vi "Sync To Server.vi"(8 "error in (no error)":errorcluster, 9 "Station":string="LTS-01", 10 "Connection String":string="Provider=MSOLEDBSQL;Data Source=.\\SQLEXPRESS;Initial Catalog=LTS;Integrated Security=SSPI;TrustServerCertificate=Yes;", 11 "DB Path":path) -> (0 "error out":errorcluster, 3 "Runs Synced":i32)   [LabVIEW 2026]
uses:
  <vilib>/drjdpowell/SQLite Library/SQL Connection/Open (path).vi
  <vilib>/drjdpowell/SQLite Library/SQL Connection/Open (string).vi
  <vilib>/AdvancedString/Path To Command Line String.vi
  <vilib>/drjdpowell/SQLite Library/SQL Connection/Execute SQL.vi
  <vilib>/addons/database/Connection.llb/DB Tools Open Connec (String).vi
  <vilib>/addons/database/Command.llb/Cmd Set Parameter Value (C).vi
  <vilib>/addons/database/Command.llb/Cmd Execute.vi
  <vilib>/addons/database/Recordset.llb/Rec Fetch Recordset Data (CR).vi
  <vilib>/addons/database/Recordset.llb/Rec Destroy - Command.vi
  <vilib>/drjdpowell/SQLite Library/SQL Connection/Execute SQL (No results).vi
  <vilib>/addons/database/Command.llb/Cmd Delete.vi
  <vilib>/drjdpowell/SQLite Library/SQL Connection/Connection.lvclass
  <vilib>/drjdpowell/SQLite Library/SQLite.lvlib
  <vilib>/addons/database/NI_Database_API.lvlib
panel:
  out "Result Set":string[][](table) caption="Result Set (from first statement with results)"
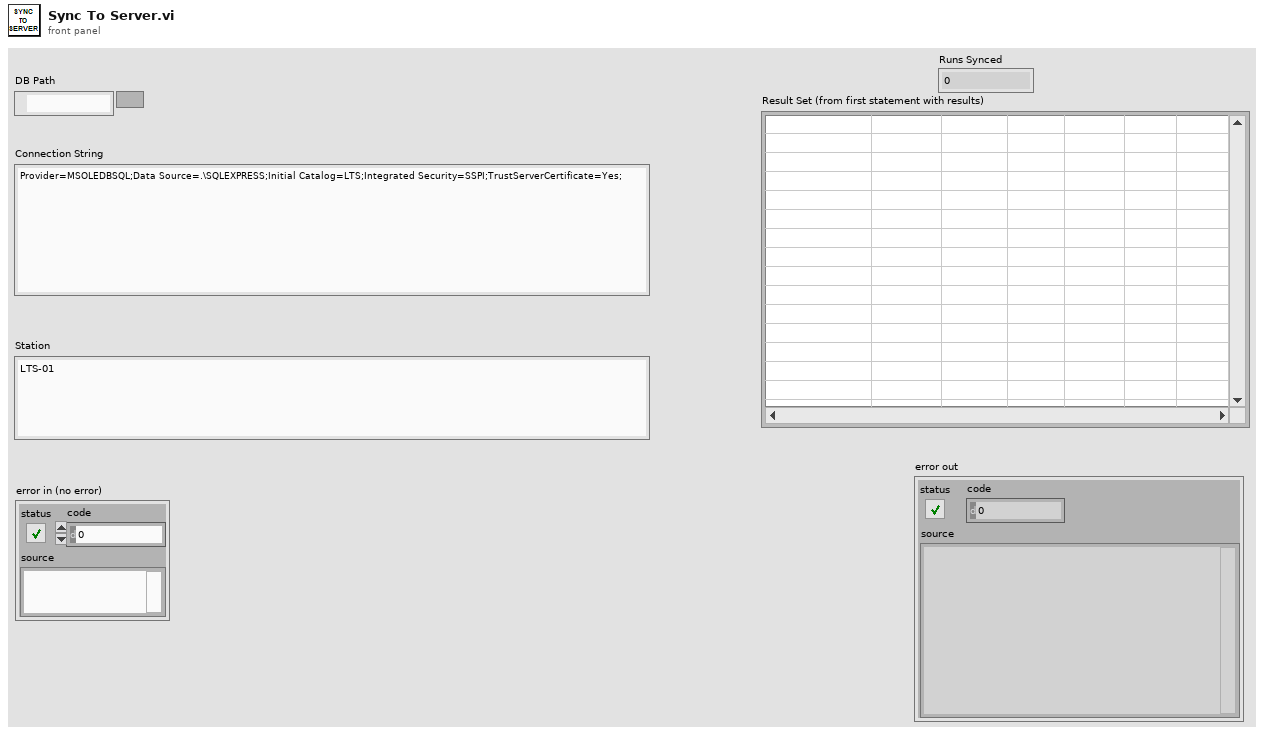
[diagram p1: front panel]
types:
  T1 = typedef "NI_Database_API.lvlib/Conn ObjectReference.ctl" = refnum<k1>
  T2 = typedef "NI_Database_API.lvlib/Cmd ObjectReference.ctl" = refnum<k1>
  T3 = typedef "NI_Database_API.lvlib/Cmd-Rec Object Reference.ctl" = refnum<k1>
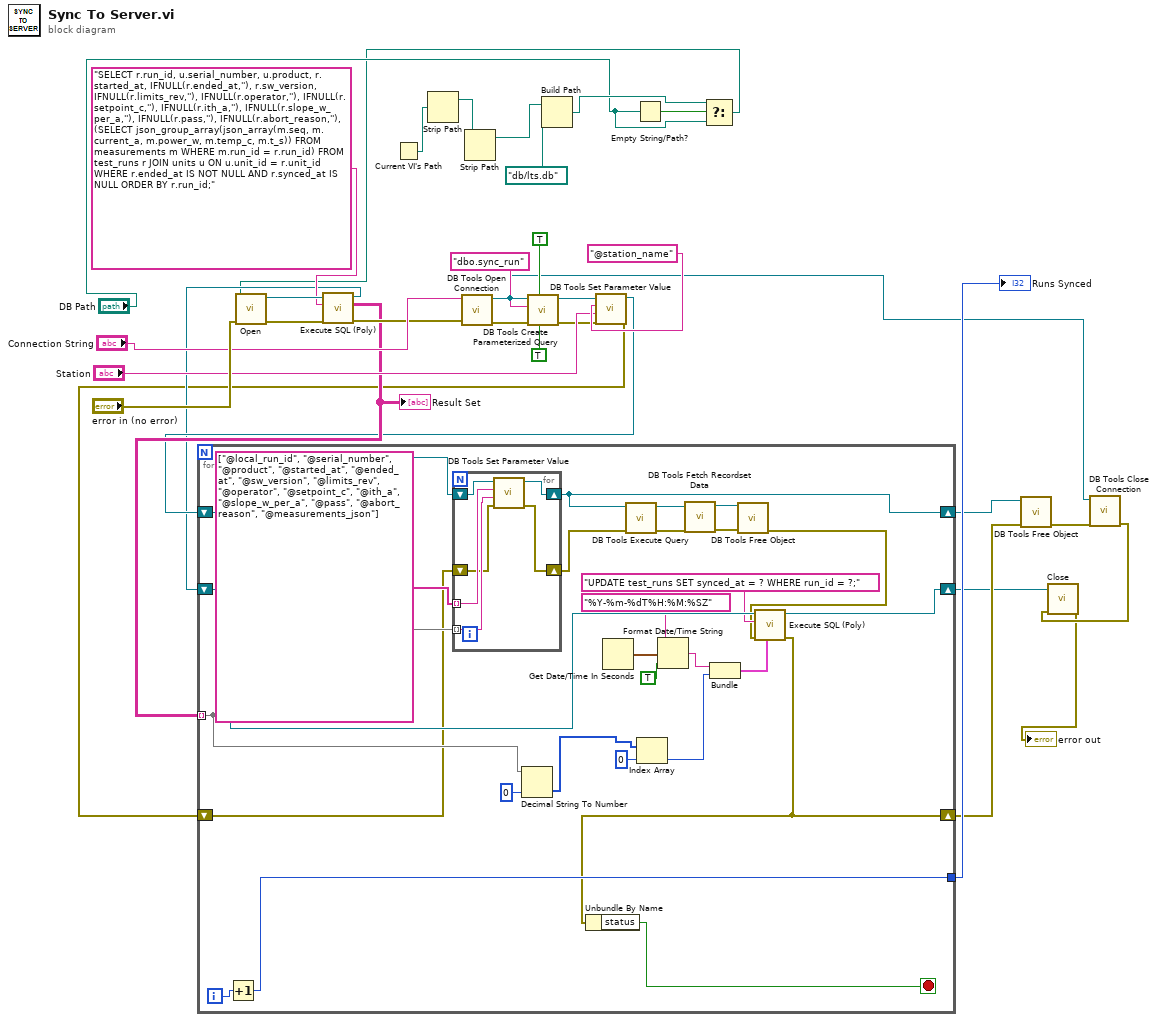
[diagram p0: block diagram]
diagram:
  n1 = Current VI's Path() -> (path=w8:path)
  n2 = Strip Path(path=w8) -> (stripped path=w7:path)  [unwired: 1 out]
  n3 = Strip Path(path=w7) -> (stripped path=w6:path)  [unwired: 1 out]
  n4 = Build Path(base path=w6, name or relative path=path "db/lts.db") -> (appended path=w3:path)
  n5 = Empty String/Path?(string/path="DB Path") -> (empty?=w4:bool)
  n6 = Select(t=w3, s=w4, f="DB Path") -> (s? t:f=w1:path)
  n7 = call-poly <vilib>:"Open.vi"("error in (no error)"="error in (no error)", "db file"=w1) -> ("error out"=w24:errorcluster, "SQLite Connection"=w33:refnum<class "Connection.lvclass">)  [unwired: 8 in]
  n8 = call-poly <vilib>:"Execute SQL (Poly).vi"("error in (no error)"=w24, "SQL"="SELECT r.run_id, u.serial_number, u.product, r.started_at, IFNULL(r.ended_at,''), r.sw_version, IFNULL(r.limits_rev,''), IFNULL(r.operator,''), IFNULL(r.setpoint_c,''), IFNULL(r.ith_a,''), IFNULL(r.slope_w_per_a,''), IFNULL(r.pass,''), IFNULL(r.abort_reason,''), (SELECT json_group_array(json_array(m.seq, m.current_a, m.power_w, m.temp_c, m.t_s)) FROM measurements m WHERE m.run_id = r.run_id) FROM test_runs r JOIN units u ON u.unit_id = r.unit_id WHERE r.ended_at IS NOT NULL AND r.synced_at IS NULL ORDER BY r.run_id;", "SQLite Connection in"=w33) -> ("error out"=w23:errorcluster, "Result Set"=w20:string[][], "SQLite Connection"=w18:refnum<class "Connection.lvclass">)  [unwired: 5 in, 1 out]
  "Result Set" <- w20
  n9 = call-poly <vilib>:"DB Tools Open Connection.vi"("error in (no error)"=w23, "connection information"="Connection String") -> ("error out"=w22:errorcluster, "connection reference"=w13:T1)  [unwired: 6 in]
  n10 = call <vilib>:"DB Tools Create Parameterized Query.vi"("stored procedure? (F)"=TRUE, "auto-detect parameters? (F)"=TRUE, "error in (no error)"=w22, "SQL query"="dbo.sync_run", "connection reference"=w13) -> ("error out"=w21:errorcluster, "command reference"=w27:T2)  [unwired: 2 in, 1 out]
  n11 = call-poly <vilib>:"DB Tools Set Parameter Value.vi"("error in (no error)"=w21, "value"="Station", "parameter index"="@station_name", "command reference"=w27) -> ("error out"=w17:errorcluster, "command reference out"=w19:T2)  [unwired: 4 in]
  n12 = for {
    tunnel: w20 -> [w39] mode=indexing
    shift-right: [w58] -> w9
    shift-left: w19 -> [w60]
    shift-right: [w40] -> w12
    shift-left: w18 -> [w53]
    shift-right: [w35] -> w15
    shift-left: w17 -> [w36]
    tunnel: [w41] -> w16
    i -> [w42]
    stop <- w59 stop-if-true
    n13 = Increment(x=w42) -> (x+1=w41:i32)
    n14 = for {
      tunnel: w39 -> [w67] mode=indexing
      shift-right: [w62] -> w58
      shift-left: w60 -> [w63]
      shift-right: [w64] -> w43
      shift-left: w36 -> [w65]
      tunnel: string[] ["@local_run_id", "@serial_number", "@product", "@started_at", "@ended_at", "@sw_version", "@limits_rev", "@operator", "@setpoint_c", "@ith_a", "@slope_w_per_a", "@pass", "@abort_reason", "@measurements_json"] -> [w66] mode=indexing
      n15 = call-poly <vilib>:"DB Tools Set Parameter Value.vi"("error in (no error)"=w65, "value"=w67, "parameter index"=w66, "command reference"=w63) -> ("error out"=w64:errorcluster, "command reference out"=w62:T2)  [unwired: 4 in]
    }
    n16 = Decimal String To Number(string=w39, default (0L)=i64 0 ("default (0 I32)")) -> (number=w37:i64[])  [unwired: 1 in, 1 out]
    n17 = Get Date/Time In Seconds() -> (seconds since 1Jan1904=w51:timestamp)
    n18 = call-poly <vilib>:"DB Tools Execute Query.vi"("error in (no error)"=w43, "command reference"=w58) -> ("error out"=w57:errorcluster, "command-recordset reference"=w56:T3)  [unwired: 6 in]
    n19 = Index Array(array=w37, index=i64 0) -> (element=w45:i64)
    n20 = Format Date/Time String(time format string (%c)="%Y-%m-%dT%H:%M:%SZ", seconds (now)=w51, UTC format=TRUE) -> (date/time string=w46:string)
    n21 = call-poly <vilib>:"DB Tools Fetch Recordset Data.vi"("error in (no error)"=w57, "command-recordset reference"=w56) -> ("error out"=w55:errorcluster, "command-recordset reference out"=w54:T3)  [unwired: 3 in, 1 out]
    n22 = Bundle(w46, w45) -> (w44:cluster{string, i64})  [unwired: 1 in]
    n23 = call-poly <vilib>:"DB Tools Free Object.vi"("error in (no error)"=w55, "command-recordset reference"=w54) -> ("error out"=w47:errorcluster)  [unwired: 8 in, 1 out]
    n24 = call-poly <vilib>:"Execute SQL (Poly).vi"("Parameter(s)"=w44, "error in (no error)"=w47, "SQL"="UPDATE test_runs SET synced_at = ? WHERE run_id = ?;", "SQLite Connection in"=w53) -> ("error out"=w35:errorcluster, "SQLite Connection"=w40:refnum<class "Connection.lvclass">)  [unwired: 6 in]
    n25 = Unbundle By Name(w35) -> ("status"=w59:bool)
  }
  "Runs Synced" <- w16
  n26 = call-poly <vilib>:"DB Tools Free Object.vi"("error in (no error)"=w15, "command reference"=w9) -> ("error out"=w14:errorcluster)  [unwired: 8 in, 1 out]
  n27 = call <vilib>:"DB Tools Close Connection.vi"("error in (no error)"=w14, "connection reference"=w13) -> ("error out"=w11:errorcluster)  [unwired: 5 in]
  n28 = call-dynamic "Close.vi"("error in (no error)"=w11, "SQLite Connection in"=w12) -> ("error out"=→"error out":errorcluster)  [unwired: 9 in]
